vi "Q calculation.vi"(6 "Correction Factor":dbl format="%#_13g", 8 "Presure psi":dbl, 10 "WB Temp":dbl, 11 "DB Temp":dbl) -> (0 "Specific Volume":dbl, 1 "Enthalpy":dbl, 2 "Relative Humidity":dbl, 3 "Humidty Ratio":dbl)   [LabVIEW 2025]
panel:
  out "pt inHg":dbl
  out "APinHg":dbl
  out "pa":dbl
  out "ps":dbl
  out "alpha":dbl
  out "pw":dbl
  out "W":dbl
  out "wdenom":dbl
  out "wnom":dbl
  out "wsat":dbl
  out "pws":dbl
  out "RT":dbl
  out "error out":errorcluster
  in  "error in":errorcluster
  in  "Presure @ Point":dbl
  in  "DB Temp":dbl
  in  "WB Temp":dbl
  out "Specific Volum":dbl
  out "h (Enthalpy)":dbl
  out "Humidity Ratio":dbl
  out "Dew Point":dbl
  out "pt":dbl
  out "Relative Humidity":dbl
  in  "ElevInFt":dbl
  # "Mathscript code"
  # "LABVIEW code"
  # "F"
  # "psi"
  # "F"
  # "psi"
  # "F"
  # "F"
  # "%"
  # "F"
  # "ft3/lbm"
  # "Btu/lbm"
  # "psi"
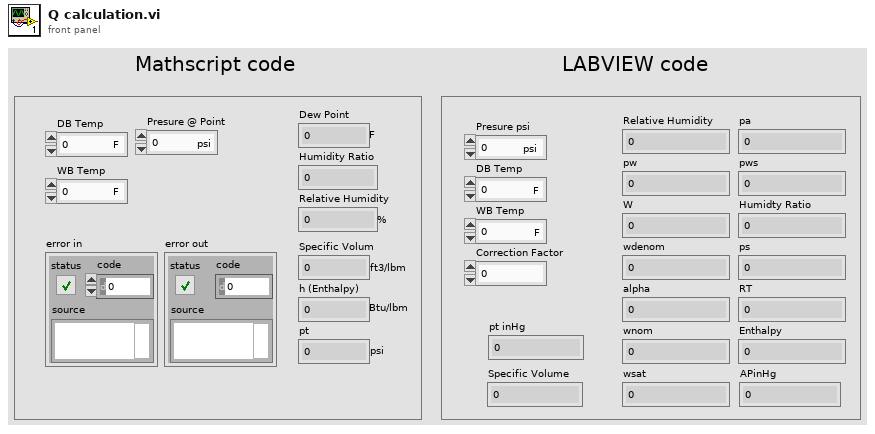
[diagram p1: front panel]
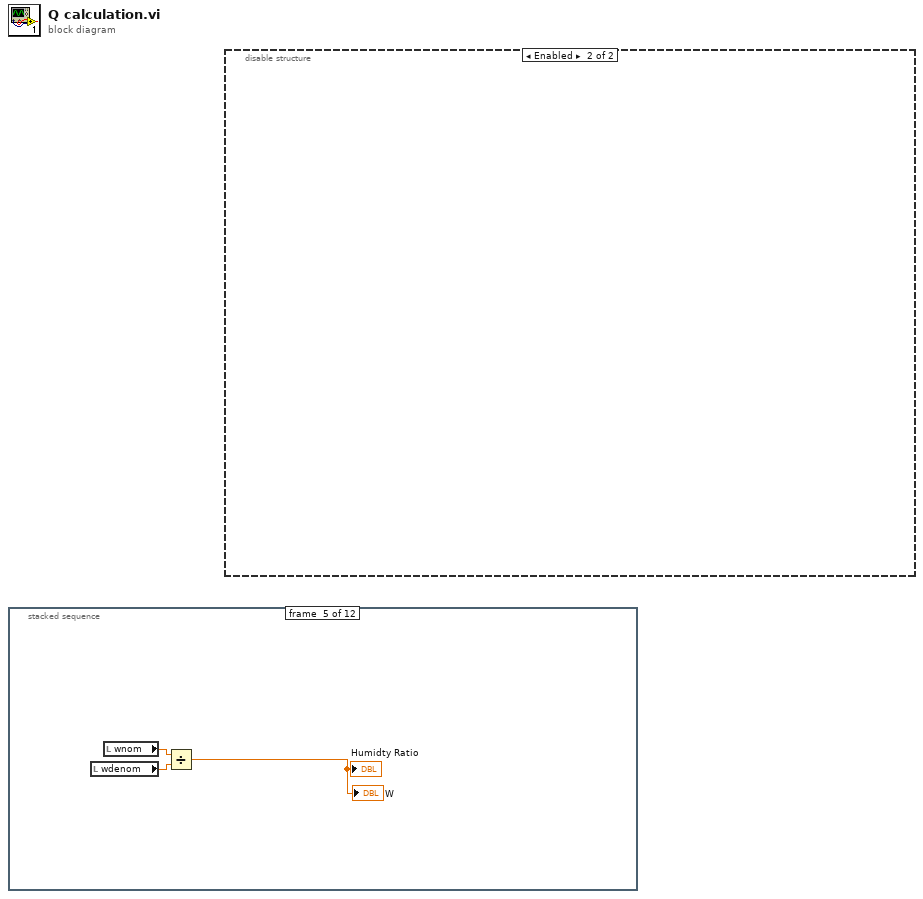
[diagram p0: block diagram]
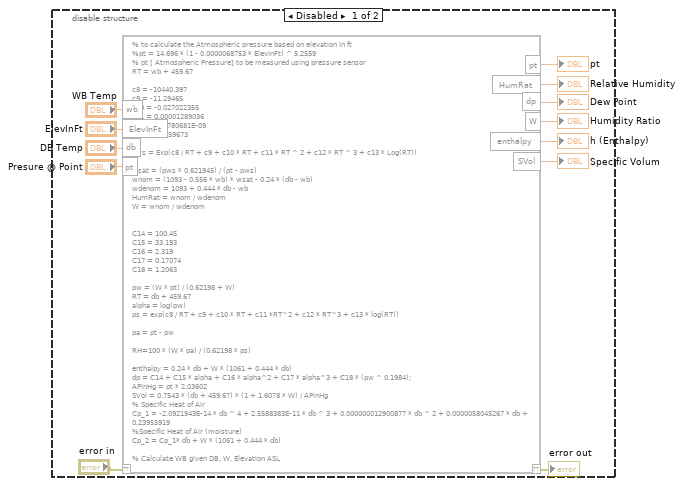
[diagram p2: hidden frame]
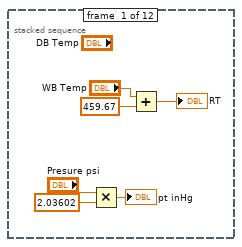
[diagram p3: hidden frame]
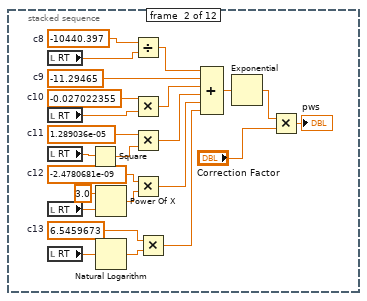
[diagram p4: hidden frame]
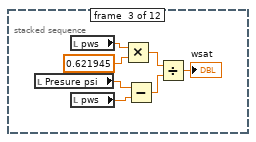
[diagram p5: hidden frame]
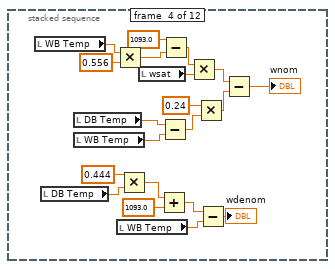
[diagram p6: hidden frame]
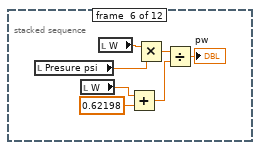
[diagram p7: hidden frame]
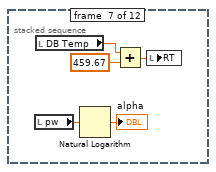
[diagram p8: hidden frame]
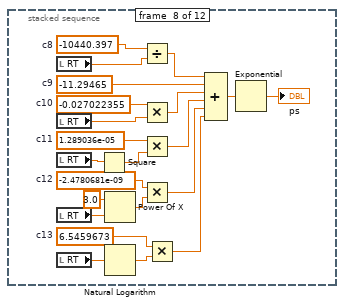
[diagram p9: hidden frame]
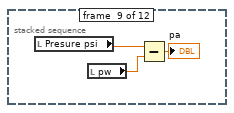
[diagram p10: hidden frame]
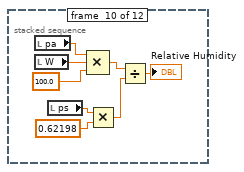
[diagram p11: hidden frame]
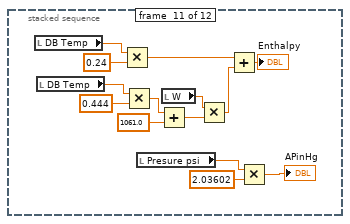
[diagram p12: hidden frame]
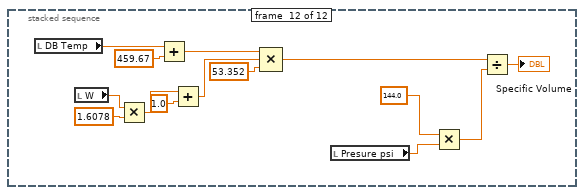
[diagram p13: hidden frame]
diagram:
  n1 = stacked-sequence {
    frame #0 {
      n2 = Multiply(x="Presure psi", y=2.03602) -> (x*y=→"pt inHg":dbl)
      n3 = Add(x="WB Temp", y=459.67) -> (x+y=→"RT":dbl)
    }
    frame #1 {
      w16 = 6.5459673  # c13
      w15 = -2.4780681e-09  # c12
      w12 = 1.289036e-05  # c11
      w11 = -0.027022355  # c10
      w13 = -11.29465  # c9
      w10 = -10440.397  # c8
      n4 = local read "RT"() -> (w30:dbl)
      n5 = local read "RT"() -> (w17:dbl)
      n6 = local read "RT"() -> (w19:dbl)
      n7 = local read "RT"() -> (w21:dbl)
      n8 = local read "RT"() -> (w23:dbl)
      n9 = Square(x=w19) -> (x^2=w18:dbl)
      n10 = Power Of X(1:w21, 2:3.0 ("y")) -> (0:w22:dbl)
      n11 = Natural Logarithm(1:w23) -> (0:w24:dbl)
      n12 = Divide(x=w10, y=w30) -> (x/y=w25:dbl)
      n13 = Multiply(x=w11, y=w17) -> (x*y=w26:dbl)
      n14 = Multiply(x=w12, y=w18) -> (x*y=w27:dbl)
      n15 = Multiply(x=w15, y=w22) -> (x*y=w28:dbl)
      n16 = Multiply(x=w16, y=w24) -> (x*y=w29:dbl)
      n17 = Compound Arithmetic op=ADD(w25, w13, w26, w27, w28, w29) -> (w20:dbl)
      n18 = Exponential(1:w20) -> (0:w8:dbl)
      n19 = Multiply(x=w8, y="Correction Factor") -> (x*y=→"pws":dbl)
    }
    frame #2 {
      n20 = local read "Presure psi"() -> (w31:dbl)
      n21 = local read "pws"() -> (w33:dbl)
      n22 = local read "pws"() -> (w34:dbl)
      n23 = Multiply(x=w33, y=0.621945) -> (x*y=w35:dbl)
      n24 = Subtract(x=w31, y=w34) -> (x-y=w36:dbl)
      n25 = Divide(x=w35, y=w36) -> (x/y=→"wsat":dbl)
    }
    frame #3 {
      n26 = local read "WB Temp"() -> (w57:dbl)
      n27 = local read "DB Temp"() -> (w42:dbl)
      n28 = local read "DB Temp"() -> (w52:dbl)
      n29 = local read "WB Temp"() -> (w51:dbl)
      n30 = Multiply(x=w57, y=0.556) -> (x*y=w56:dbl)
      n31 = local read "WB Temp"() -> (w41:dbl)
      n32 = Multiply(x=0.444 ("y"), y=w42) -> (x*y=w40:dbl)
      n33 = local read "wsat"() -> (w54:dbl)
      n34 = Add(x=w40, y=1093.0) -> (x+y=w43:dbl)
      n35 = Subtract(x=w52, y=w51) -> (x-y=w50:dbl)
      n36 = Subtract(x=1093.0, y=w56) -> (x-y=w55:dbl)
      n37 = Multiply(x=w55, y=w54) -> (x*y=w53:dbl)
      n38 = Multiply(x=0.24 ("y"), y=w50) -> (x*y=w49:dbl)
      n39 = Subtract(x=w43, y=w41) -> (x-y=→"wdenom":dbl)
      n40 = Subtract(x=w53, y=w49) -> (x-y=→"wnom":dbl)
    }
    frame #4 {
      n41 = local read "wdenom"() -> (w60:dbl)
      n42 = local read "wnom"() -> (w59:dbl)
      n43 = Divide(x=w59, y=w60) -> (x/y=→"Humidty Ratio" →"W":dbl)
    }
    frame #5 {
      n44 = local read "Presure psi"() -> (w67:dbl)
      n45 = local read "W"() -> (w64:dbl)
      n46 = local read "W"() -> (w66:dbl)
      n47 = Add(x=w64, y=0.62198) -> (x+y=w62:dbl)
      n48 = Multiply(x=w66, y=w67) -> (x*y=w65:dbl)
      n49 = Divide(x=w65, y=w62) -> (x/y=→"pw":dbl)
    }
    frame #6 {
      n50 = local read "pw"() -> (w69:dbl)
      n51 = local read "DB Temp"() -> (w70:dbl)
      n52 = Natural Logarithm(1:w69) -> (0:→"alpha":dbl)
      n53 = Add(x=w70, y=459.67) -> (x+y=w71:dbl)
      n54 = local write "RT"(w71) -> ()
    }
    frame #7 {
      w79 = 6.5459673  # c13
      w78 = -2.4780681e-09  # c12
      w75 = 1.289036e-05  # c11
      w74 = -0.027022355  # c10
      w76 = -11.29465  # c9
      w73 = -10440.397  # c8
      n55 = local read "RT"() -> (w94:dbl)
      n56 = local read "RT"() -> (w80:dbl)
      n57 = local read "RT"() -> (w82:dbl)
      n58 = local read "RT"() -> (w84:dbl)
      n59 = local read "RT"() -> (w86:dbl)
      n60 = Square(x=w82) -> (x^2=w81:dbl)
      n61 = Power Of X(1:w84, 2:3.0 ("y")) -> (0:w85:dbl)
      n62 = Natural Logarithm(1:w86) -> (0:w87:dbl)
      n63 = Divide(x=w73, y=w94) -> (x/y=w88:dbl)
      n64 = Multiply(x=w74, y=w80) -> (x*y=w89:dbl)
      n65 = Multiply(x=w75, y=w81) -> (x*y=w90:dbl)
      n66 = Multiply(x=w78, y=w85) -> (x*y=w91:dbl)
      n67 = Multiply(x=w79, y=w87) -> (x*y=w92:dbl)
      n68 = Compound Arithmetic op=ADD(w88, w76, w89, w90, w91, w92) -> (w83:dbl)
      n69 = Exponential(1:w83) -> (0:→"ps":dbl)
    }
    frame #8 {
      n70 = local read "Presure psi"() -> (w97:dbl)
      n71 = local read "pw"() -> (w96:dbl)
      n72 = Subtract(x=w97, y=w96) -> (x-y=→"pa":dbl)
    }
    frame #9 {
      n73 = local read "pa"() -> (w105:dbl)
      n74 = local read "W"() -> (w104:dbl)
      n75 = local read "ps"() -> (w102:dbl)
      n76 = Compound Arithmetic op=MULTIPLY(w105, w104, 100.0 ("value")) -> (w100:dbl)
      n77 = Multiply(x=w102, y=0.62198) -> (x*y=w99:dbl)
      n78 = Divide(x=w100, y=w99) -> (x/y=→"Relative Humidity":dbl)
    }
    frame #10 {
      n79 = local read "DB Temp"() -> (w119:dbl)
      n80 = local read "DB Temp"() -> (w116:dbl)
      n81 = Multiply(x=w119, y=0.24) -> (x*y=w110:dbl)
      n82 = Multiply(x=w116, y=0.444) -> (x*y=w115:dbl)
      n83 = local read "Presure psi"() -> (w107:dbl)
      n84 = Add(x=w115, y=1061.0) -> (x+y=w113:dbl)
      n85 = local read "W"() -> (w112:dbl)
      n86 = Multiply(x=w112, y=w113) -> (x*y=w111:dbl)
      n87 = Add(x=w110, y=w111) -> (x+y=→"Enthalpy":dbl)
      n88 = Multiply(x=w107, y=2.03602) -> (x*y=→"APinHg":dbl)
    }
    frame #11 {
      n89 = local read "DB Temp"() -> (w132:dbl)
      n90 = local read "W"() -> (w130:dbl)
      n91 = Multiply(x=w130, y=1.6078) -> (x*y=w128:dbl)
      n92 = Add(x=w132, y=459.67) -> (x+y=w126:dbl)
      n93 = Add(x=w128, y=1.0) -> (x+y=w125:dbl)
      n94 = Compound Arithmetic op=MULTIPLY(w126, w125, 53.352 ("value")) -> (w123:dbl)
      n95 = local read "Presure psi"() -> (w120:dbl)
      n96 = Multiply(x=144.0, y=w120) -> (x*y=w122:dbl)
      n97 = Divide(x=w123, y=w122) -> (x/y=→"Specific Volume":dbl)
    }
  }
  n98 = disable-structure shown="Enabled" {
    frame Disabled {
      n99 = mathscript code="% to calculate the Atmospheric pressure based on elevation in ft\n%pt = 14.696 * (1 - 0.0000068753 * ElevInFt) ^ 5.2559   \n% pt [ Atmospheric Pressure] to be measured using pressure sensor\nRT = wb + 459.67\n\nc8 = -10440.397\nc9 = -11.29465\nc10 = -0.027022355\nc11 = 0.00001289036\nc12 = -2.4780681E-09\nc13 = 6.5459673\n\npws = Exp(c8 / RT + c9 + c10 * RT + c11 * RT ^ 2 + c12 * RT ^ 3 + c13 * Log(RT))\n\nwsat = (pws * 0.621945) / (pt - pws)\nwnom = (1093 - 0.556 * wb) * wsat - 0.24 * (db - wb)\nwdenom = 1093 + 0.444 * db - wb\nHumRat = wnom / wdenom\nW = wnom / wdenom\n\n\nC14 = 100.45\nC15 = 33.193\nC16 = 2.319\nC17 = 0.17074\nC18 = 1.2063\n\npw = (W * pt) / (0.62198 + W)\nRT = db + 459.67\nalpha = log(pw)\nps = exp(c8 / RT + c9 + c10 * RT + c11 *RT^2 + c12 * RT^3 + c13 * log(RT))\n\npa = pt - pw\n\nRH=100 * (W * pa) / (0.62198 * ps)\n\nenthalpy = 0.24 * db + W * (1061 + 0.444 * db)\ndp = C14 + C15 * alpha + C16 * alpha^2 + C17 * alpha^3 + C18 * (pw ^ 0.1984);\nAPinHg = pt * 2.03602\nSVol = 0.7543 * (db + 459.67) * (1 + 1.6078 * W) / APinHg\n% Specific Heat of Air\nCp_1 = -2.0921943E-14 * db ^ 4 + 2.5588383E-11 * db ^ 3 + 0.000000012900877 * db ^ 2 + 0.0000058045267 * db + 0.23955919\n%Specific Heat of Air (moisture)\nCp_2 = Cp_1* db + W * (1061 + 0.444 * db)\n\n% Calculate WB given DB, W, Elevation ASL"("??"="error in", "wb"="WB Temp", "ElevInFt"="ElevInFt", "db"="DB Temp", "pt"="Presure @ Point") -> ("??"=→"error out":errorcluster, "HumRat"=→"Relative Humidity":dbl, "pt"=→"pt":dbl, "W"=→"Humidity Ratio":cdb, "enthalpy"=→"h (Enthalpy)":cdb, "dp"=→"Dew Point":cdb, "SVol"=→"Specific Volum":cdb)
    }
    frame Enabled {
    }
  }
